vi "Test Runner Pre-build action.vi"(6 "Top Level/Always Included VIs":path[](array[path]), 7 "Main Destination Path":path, 9 "Target Name":string, 10 "Build Specification Name":string, 11 "Project Path":path) -> (0 "error out":errorcluster)   [LabVIEW 2020]
uses:
  classes/Test Report.JUnit/Test Report.JUnit.lvclass
  C:/projects/caraya/src/classes/Test Report/Test Report.lvclass
  classes/Test Runner.Folder/Test Runner.Folder.lvclass
  C:/projects/caraya/src/classes/Test Runner/Test Runner.lvclass
  classes/Test Runner/Test Runner.lvclass
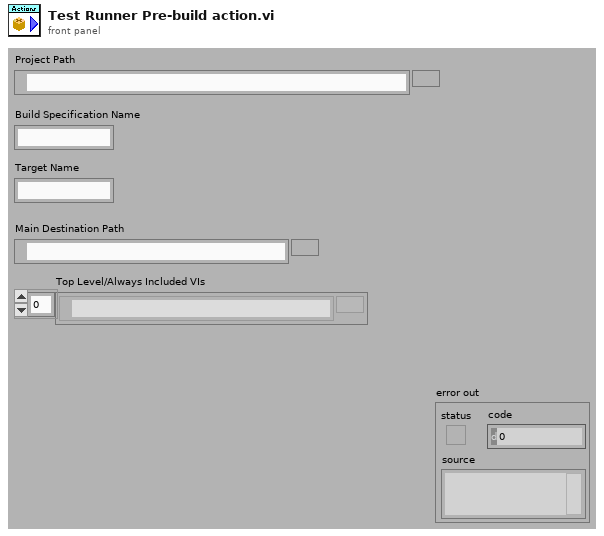
[diagram p1: front panel]
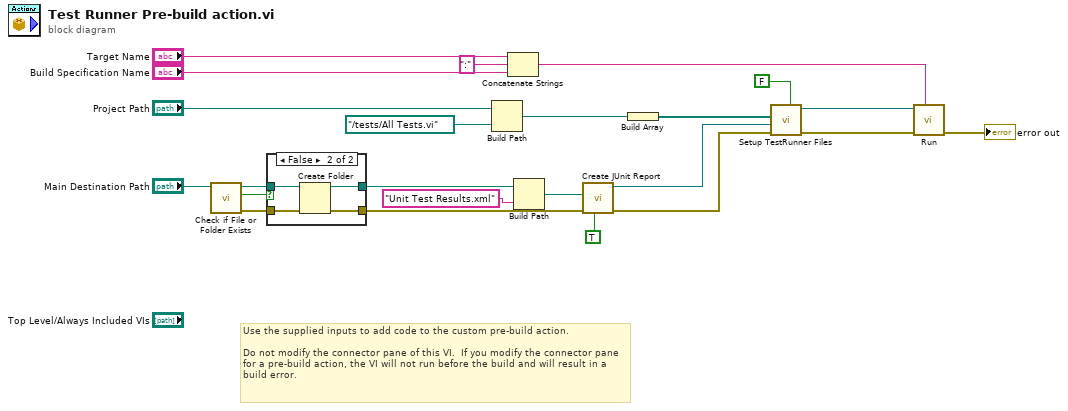
[diagram p0: block diagram]
diagram:
  # "Use the supplied inputs to add code to the custom pre-build action.\n\nDo not modify the connector pane of this VI.  If you modify the connector pane for a pre-build action, the VI will not run before the build and will result in a build error."
  n1 = call <vilib>:"Check if File or Folder Exists.vi"("path"="Main Destination Path") -> ("error out"=w15:errorcluster, "file or folder exists?"=w16:bool, "dup path"=w18:path)  [unwired: 8 in]
  n2 = case shown="False" w16 {
    tunnel: w18 -> [w25 w29]
    tunnel: [w25 w28] -> w17
    tunnel: w15 -> [w24 w27]
    tunnel: [w24 w26] -> w12
    frame True {
    }
    frame False {
      n3 = Create Folder(path (use dialog)=w29, error in=w27) -> (created path=w28:path, error out=w26:errorcluster)  [unwired: 1 in, 1 out]
    }
  }
  n4 = Build Path(base path="Project Path", name or relative path=path "../tests/All Tests.vi" ("Test VI")) -> (appended path=w7:path)
  n5 = Concatenate Strings("Target Name", ":" ("string"), "Build Specification Name") -> (w11:string)
  n6 = Build Path(base path=w17, name or relative path="Unit Test Results.xml") -> (appended path=w14:path)
  n7 = call "Create JUnit Report.vi"("Verbose"=TRUE, "error in (no error)"=w12, "Report Path"=w14) -> ("error out"=w1:errorcluster, "Test Report.JUnit out"=w4:refnum<class "Test Report.JUnit.lvclass">)  [unwired: 7 in]
  n8 = Build Array(w7) -> (w6:path[])
  n9 = call "Setup TestRunner Files.vi"("Interactive (T)"=FALSE, "error in (no error)"=w1, "Test Report"=w4, "Paths"=w6) -> ("error out"=w3:errorcluster, "Test Runner.Folder out"=w2:refnum<class "Test Runner.Folder.lvclass">)  [unwired: 6 in]
  n10 = call "Run.vi"("Name"=w11, "error in (no error)"=w3, "Test Runner in"=w2) -> ("error out"=→"error out":errorcluster)  [unwired: 6 in, 2 out]
